vi "Two Way Event Recorder Init RS232 Comms.vi"(8 "error in (no error)":errorcluster, 11 "Device Ref in":T1 format="%.0x") -> (0 "error out":errorcluster, 3 "Visa reference out":refnum<visa-resource-name>)   [LabVIEW 2017, in "Two Way Event Recorder Custom Device.lvlib"]
uses:
  Two Way Event Recorder Custom Device.lvlib
  <vilib>/NI Veristand/Custom Device API/Custom Device Item Ref.ctl
  Two Way Event Recorder Property Lookup.vi
  <vilib>/NI Veristand/Custom Device API/Get Item Property (String).vi
  <vilib>/NI Veristand/Custom Device API/Get Item Property (U32).vi
  <vilib>/NI Veristand/Custom Device API/Get Item Property (U16).vi
  <vilib>/NI Veristand/Custom Device API/Custom Device API.lvlib
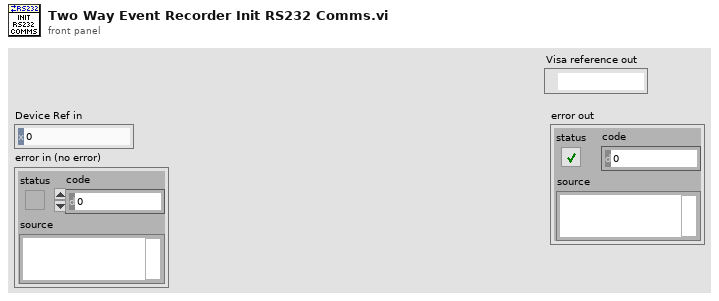
[diagram p1: front panel]
types:
  T1 = typedef "Custom Device API.lvlib/Custom Device Item Ref.ctl" = u64
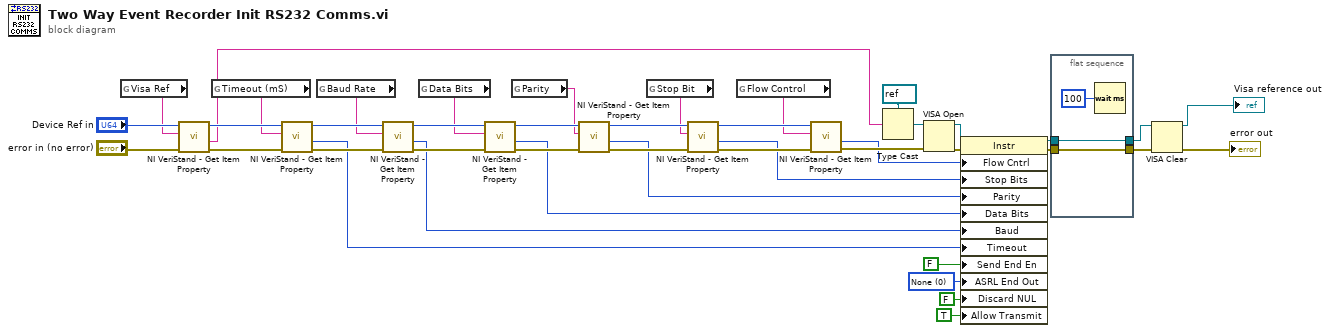
[diagram p0: block diagram]
diagram:
  w3 = u16 0 items=["None", "Last Bit", "TermChar", "Break"] ("Serial Settings:End Mode for Writes")
  n1 = global read "Two Way Event Recorder Property Lookup.vi" "Visa Ref"() -> (w17:string)
  n2 = call-poly <vilib>:"NI VeriStand - Get Item Property.vi"("error in (no error)"="error in (no error)", "Property Name"=w17, "Item Ref in"="Device Ref in") -> ("error out"=w41:errorcluster, "Value"=w30:string, "Item Ref out"=w43:T1)  [unwired: 5 in, 1 out]
  n3 = global read "Two Way Event Recorder Property Lookup.vi" "Timeout (mS)"() -> (w16:string)
  n4 = call-poly <vilib>:"NI VeriStand - Get Item Property.vi"("error in (no error)"=w41, "Property Name"=w16, "Item Ref in"=w43) -> ("error out"=w39:errorcluster, "Value"=w20:u32, "Item Ref out"=w42:T1)  [unwired: 5 in, 1 out]
  n5 = global read "Two Way Event Recorder Property Lookup.vi" "Baud Rate"() -> (w15:string)
  n6 = call-poly <vilib>:"NI VeriStand - Get Item Property.vi"("error in (no error)"=w39, "Property Name"=w15, "Item Ref in"=w42) -> ("error out"=w38:errorcluster, "Value"=w21:u32, "Item Ref out"=w40:T1)  [unwired: 5 in, 1 out]
  n7 = global read "Two Way Event Recorder Property Lookup.vi" "Data Bits"() -> (w14:string)
  n8 = call-poly <vilib>:"NI VeriStand - Get Item Property.vi"("error in (no error)"=w38, "Property Name"=w14, "Item Ref in"=w40) -> ("error out"=w37:errorcluster, "Value"=w22:u16, "Item Ref out"=w36:T1)  [unwired: 5 in, 1 out]
  n9 = global read "Two Way Event Recorder Property Lookup.vi" "Parity"() -> (w13:string)
  n10 = call-poly <vilib>:"NI VeriStand - Get Item Property.vi"("error in (no error)"=w37, "Property Name"=w13, "Item Ref in"=w36) -> ("error out"=w34:errorcluster, "Value"=w23:u16, "Item Ref out"=w35:T1)  [unwired: 5 in, 1 out]
  n11 = global read "Two Way Event Recorder Property Lookup.vi" "Stop Bit"() -> (w12:string)
  n12 = call-poly <vilib>:"NI VeriStand - Get Item Property.vi"("error in (no error)"=w34, "Property Name"=w12, "Item Ref in"=w35) -> ("error out"=w33:errorcluster, "Value"=w24:u16, "Item Ref out"=w32:T1)  [unwired: 5 in, 1 out]
  n13 = global read "Two Way Event Recorder Property Lookup.vi" "Flow Control"() -> (w11:string)
  n14 = call-poly <vilib>:"NI VeriStand - Get Item Property.vi"("error in (no error)"=w33, "Property Name"=w11, "Item Ref in"=w32) -> ("error out"=w27:errorcluster, "Value"=w25:u16)  [unwired: 5 in, 2 out]
  n15 = Type Cast(type=refnum<visa-resource-name> refnum ("reference"), x=w30) -> (*(type *) &x=w29:refnum<visa-resource-name>)
  n16 = VISA Open(error in (no error)=w27, VISA resource name=w29) -> (VISA resource name=w26:refnum<visa-resource-name>, error out=w28:errorcluster)  [unwired: 3 in]
  n17 = property class="Instr"(reference=w26, error in=w28, "Flow Cntrl"=w25, "Stop Bits"=w24, "Parity"=w23, "Data Bits"=w22, "Baud"=w21, "Timeout"=w20, "Send End En"=FALSE ("Message Based Settings:Send End Enable"), "ASRL End Out"=w3, "Discard NUL"=FALSE ("Serial Settings:Discard NUL Characters"), "Allow Transmit"=TRUE ("Serial Settings:Allow Transmit")) -> (reference out=w9:refnum<visa-resource-name>, error out=w10:errorcluster)
  n18 = flat-sequence {
    tunnel: w10 -> [w45]
    tunnel: w9 -> [w46]
    tunnel: [w46] -> w7
    tunnel: [w45] -> w8
    frame #0 {
      n19 = Wait (ms)(milliseconds to wait=u32 100) -> ()  [unwired: 1 out]
    }
  }
  n20 = VISA Clear(VISA resource name=w7, error in (no error)=w8) -> (VISA resource name out=→"Visa reference out":refnum<visa-resource-name>, error out=→"error out":errorcluster)
